vi "GDM-9052 Read Temperature.vi"() -> ()   [LabVIEW 2021, in "GDM-9052.lvlib"]
uses:
  GDM-9052.lvlib
panel:
  in  "Configure RS232 Baud Rate":u32(ring)=115200 items=["9600"=9600, "19200"=19200, "38400"=38400, "57600"=57600, "115200"=115200]
  in  "Simulation Value":dbl=23.0 min=0.0 max=50.0 step=0.01 format="%.2f"
  in  "Temperature Unit":u16(ring) items=["C", "F"]
  in  "Type for Temperature":u16(ring) items=["J Type", "K Type", "T Type"]
  out "error out":errorcluster
  out "Measure Value":string
  in  "Stop":bool
  out "Boolean":bool
  in  "Detector Rate":u16(ring) items=["SLOW", "MID", "FAST"]
  out "ID Return String":string
  in  "VISA resource name":refnum<visa-resource-name>
  # "GDM-9052 Read Temperature"
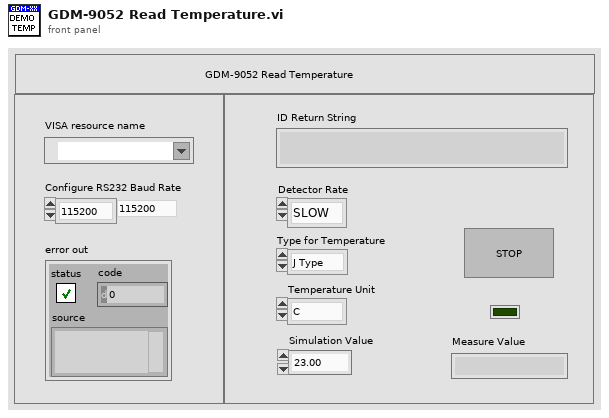
[diagram p1: front panel]
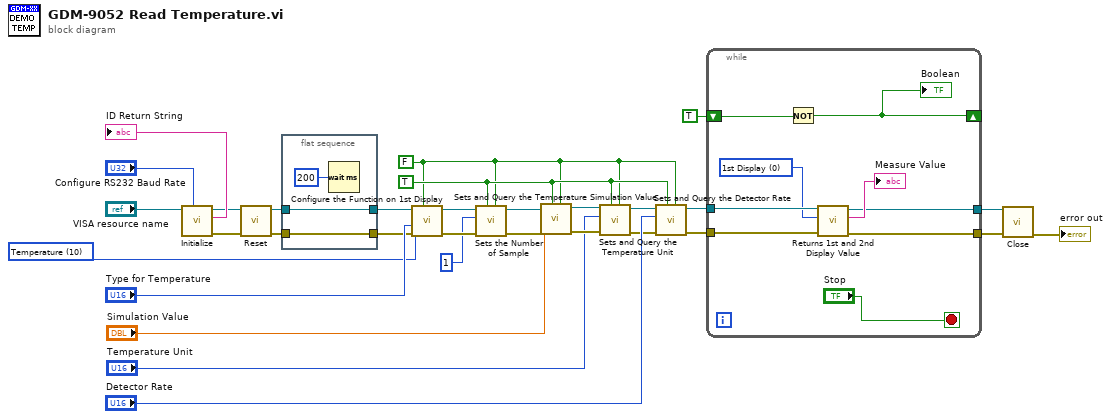
[diagram p0: block diagram]
diagram:
  w1 = u8 10 items=["DC Voltage", "AC Voltage", "DC Current", "AC Current", "2-Wire Resistance", "4-Wire Resistance", "Frequency", "Period", "Continuity", "Diode", "Temperature", "Capacitance"] ("Function")
  w6 = FALSE ("Enable to Query")
  w7 = TRUE ("Enable to Sets")
  n1 = call "Initialize.vi"("Configure RS232 Baud Rate"="Configure RS232 Baud Rate", "VISA resource name"="VISA resource name") -> ("error out"=w22:errorcluster, "ID Return String"=→"ID Return String":string, "VISA resource name out"=w23:refnum<visa-resource-name>)  [unwired: 6 in, 1 out]
  n2 = call "Reset.vi"("error in (no error)"=w22, "VISA resource name"=w23) -> ("error out"=w11:errorcluster, "VISA resource name out"=w13:refnum<visa-resource-name>)  [unwired: 8 in]
  n3 = flat-sequence {
    tunnel: w13 -> [w34]
    tunnel: [w34] -> w12
    tunnel: w11 -> [w33]
    tunnel: [w33] -> w10
    frame #0 {
      n4 = Wait (ms)(milliseconds to wait=u32 200) -> ()  [unwired: 1 out]
    }
  }
  n5 = call "Configure the Function on 1st Display .vi"("Enable Auto Range"=w6, "error in"=w10, "Type for Temperature"="Type for Temperature", "Function"=w1, "VISA resource name"=w12) -> ("error out"=w5:errorcluster, "VISA resource name out"=w9:refnum<visa-resource-name>)  [unwired: 5 in]
  n6 = call "Sets the Number of Sample.vi"("Enable to Query"=w6, "Enable to Sets"=w7, "error in"=w5, "Number of Sample"=u16 1, "VISA resource name"=w9) -> ("error out"=w4:errorcluster, "VISA resource name out"=w8:refnum<visa-resource-name>)  [unwired: 4 in, 1 out]
  n7 = call "Sets and Query the Temperature Simulation Value.vi"("Enable to Query"=w6, "Enable to Sets"=w7, "error in"=w4, "Simulation Value"="Simulation Value", "VISA resource name"=w8) -> ("error out"=w16:errorcluster, "VISA resource name out"=w17:refnum<visa-resource-name>)  [unwired: 4 in, 1 out]
  n8 = call "Sets and Query the Temperature Unit.vi"("Enable to Query"=w6, "Enable to Sets"=w7, "error in"=w16, "Temperature Unit"="Temperature Unit", "VISA resource name"=w17) -> ("error out"=w19:errorcluster, "VISA resource name out"=w18:refnum<visa-resource-name>)  [unwired: 4 in, 1 out]
  n9 = call "Sets and Query the Detector Rate.vi"("Enable to Query"=w6, "Enable to Sets"=w7, "error in"=w19, "Detector Rate"="Detector Rate", "VISA resource name"=w18) -> ("error out"=w27:errorcluster, "VISA resource name out"=w28:refnum<visa-resource-name>)  [unwired: 4 in, 1 out]
  n10 = while {
    tunnel: w28 -> [w43]
    tunnel: w27 -> [w42]
    tunnel: [w38] -> w26
    tunnel: [w37] -> w25
    shift-right: [w35] -> _
    shift-left: TRUE -> [w36]
    stop <- "Stop" stop-if-true
    w41 = u16 0 items=["1st Display", "2nd Display", "1st & 2nd Display"] ("Sets to Display")
    n11 = Not(x=w36) -> (.not. x?=w35:bool)
    "Boolean" <- w35
    n12 = call "Returns 1st and 2nd Display Value.vi"("error in"=w42, "Sets to Display"=w41, "VISA resource name"=w43) -> ("error out"=w37:errorcluster, "Return the Value"=→"Measure Value":string, "VISA resource name out"=w38:refnum<visa-resource-name>)  [unwired: 6 in]
  }
  n13 = call "Close.vi"("error in (no error)"=w25, "VISA resource name"=w26) -> ("error out"=→"error out":errorcluster)  [unwired: 9 in]
